vi "VIH Utility - UI - Key Focus & Selection Color (Listbox).vi"(5 "Selection color if inactive":u32(colorbox)=13816530, 7 "Selection color if active":u32(colorbox)=16777224, 8 "error in":errorcluster, 10 "F:Test/T:Set Key Focus (F)":bool, 11 "LstBox Refnum":refnum<vi>) -> (0 "error out":errorcluster, 1 "Key Focus?":bool, 3 "dup MCListbox Refnum":refnum<vi>)   [LabVIEW 2014]
doc: "::: VI Helpeks :::\nCopyright (c) 2000-2026 Konstantin Shifershteyn. All rights reserved."
panel:
  # "VI Helpeks\nCopyright (c) 2012-2026 Konstantin Shifershteyn"
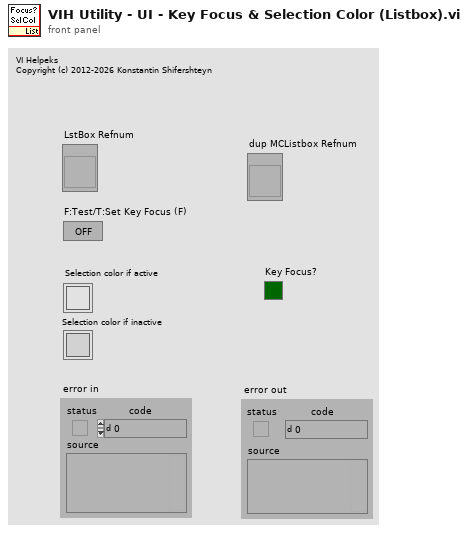
[diagram p1: front panel]
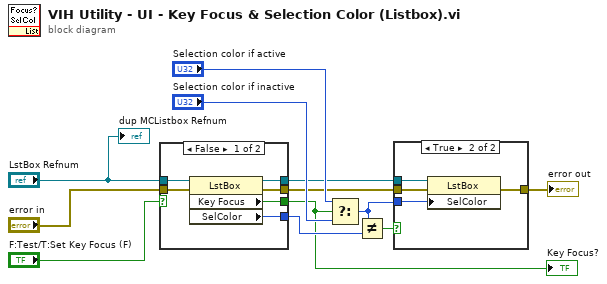
[diagram p0: block diagram]
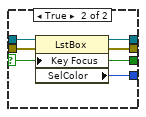
[diagram p2: hidden frame]
diagram:
  n1 = case shown="False" "F:Test/T:Set Key Focus (F)" {
    selector: "F:Test/T:Set Key Focus (F)" -> [_ w23]
    tunnel: [w18 w23] -> w1
    tunnel: [w17 w24] -> w8
    tunnel: "LstBox Refnum" -> [w16 w22]
    tunnel: "error in" -> [w15 w21]
    tunnel: [w14 w20] -> w5
    tunnel: [w13 w19] -> w4
    frame False {
      n2 = property on="Property Node" class="LstBox"(reference=w16, error in=w15) -> (reference out=w14:refnum<vi>, error out=w13:errorcluster, "Key Focus"=w18:bool, "SelColor"=w17:u32)
    }
    frame True {
      n3 = property on="Property Node" class="LstBox"(reference=w22, error in=w21, "Key Focus"=w23) -> (reference out=w20:refnum<vi>, error out=w19:errorcluster, "SelColor"=w24:u32)
    }
  }
  "Key Focus?" <- w1
  n4 = Select(t="Selection color if active", s=w1, f="Selection color if inactive") -> (s? t:f=w6:u32)
  n5 = Not Equal?(x=w6, y=w8) -> (x != y?=w7:bool)
  n6 = case shown="True" w7 {
    tunnel: w6 -> [_ w29]
    tunnel: w5 -> [_ w28]
    tunnel: w4 -> [w25 w27]
    tunnel: [w25 w26] -> w9
    frame False {
    }
    frame True {
      n7 = property on="Property Node" class="LstBox"(reference=w28, error in=w27, "SelColor"=w29) -> (error out=w26:errorcluster)  [unwired: 1 out]
    }
  }
  "error out" <- w9
  "dup MCListbox Refnum" <- "LstBox Refnum"
